vi "json.generate_object.vi"(8 "error in":errorcluster, 11 "ts.iso8601 in":refnum<class "ts.iso8601.lvclass">) -> (0 "error out":errorcluster, 2 "JSON Object":string, 3 "ts.iso8601 out":refnum<class "ts.iso8601.lvclass">)   [LabVIEW 2020, in "ts.iso8601.lvclass"]
uses:
  ts.iso8601.lvclass
  fc4585b6-f5f8-418e-b4b0-6256cccee070.vi
  <vilib>/JDP Science/JSONtext/Variant to JSON Text.vi
  <vilib>/JDP Science/JSONtext/LVClass Serializer/JSONtext LVClass Serializer.lvclass
panel:
  # "{\n\"seriesName\":\"tom\",\n\"timestampType\":{\n\"type\":absolute,\n\"absolute\":{\"type\":\"iso8601\"}\n}\n}"
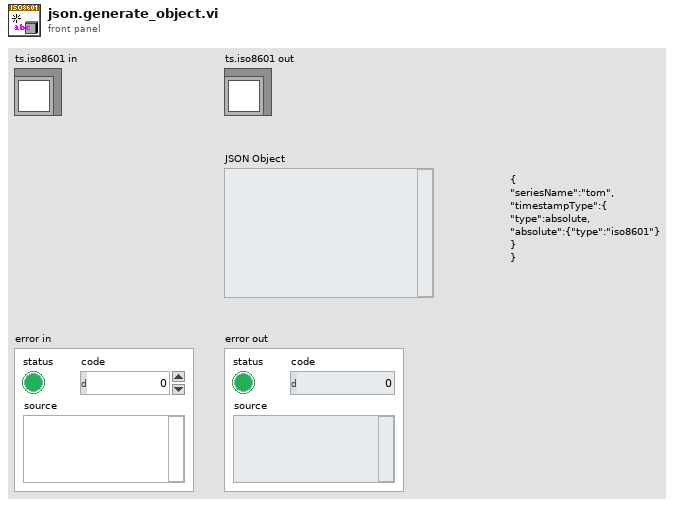
[diagram p1: front panel]
types:
  T1 = cluster{"seriesName":string, "timestampType":cluster{"type":string, "absolute":cluster{"type":string}}}
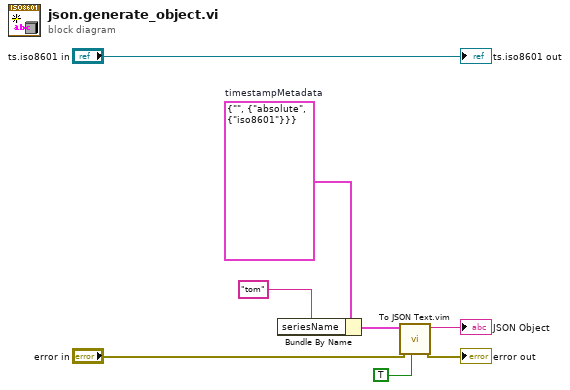
[diagram p0: block diagram]
diagram:
  w2 = T1 {"seriesName"="", "timestampType"={"type"="absolute", "absolute"={"type"="iso8601"}}}  # timestampMetadata
  n1 = Bundle By Name(cluster=w2, "seriesName"="tom") -> (w8:T1)
  n2 = call "To JSON Text.vim"("Pretty Print?"=TRUE, "error in (no error)"="error in", "Anything"=w8) -> ("error out"=→"error out":errorcluster, "<JSON>"=→"JSON Object":string)  [unwired: 7 in]
  "ts.iso8601 out" <- "ts.iso8601 in"
